vi "Single_Start_PB.vi"   [LabVIEW 2024]
uses:
  SpinCore_API_file_location.vi
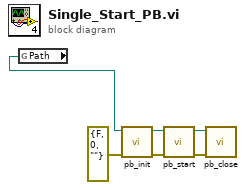
[diagram p0: block diagram]
diagram:
  n1 = global read "SpinCore_API_file_location.vi" "Path"() -> (w1:path)
  n2 = call "pb_init.vi"("error in (no error)"=errorcluster {"status"=FALSE, "code"=0, "source"=""}, "path in"=w1) -> ("error out"=w3:errorcluster, "path out"=w5:path)  [unwired: 1 in, 7 out]
  n3 = call "pb_start.vi"("error in (no error)"=w3, "path in"=w5) -> ("error out"=w2:errorcluster, "path out"=w6:path)  [unwired: 1 in, 7 out]
  n4 = call "pb_close.vi"("error in (no error)"=w2, "path in"=w6) -> ()  [unwired: 10 out]
